vi "Claude_View.vi"(0 "State":T2={"Tick"=0, "Phase"=0, "PhaseTicks"=0, "Level"=1, "Room"=0, "X10"=0, "Y10"=0, "VY10"=0, "Mode"=0, "Facing"=0, "Run"=0, "Vert"=0, "StandY"=0, "EntryX10"=0, "EntryY10"=0, "EntryMode"=0, "Lives"=4, "Score"=0, "NextLife"=10000, "KeyR"=0, "KeyB"=0, "KeyY"=0, "Torch"=FALSE, "FloorPhase"=0, "Dead"=FALSE, "LevelStart"=FALSE, "Quit"=FALSE, "Sound"=0, "Seed"=12345, "DemoStep"=0, "Tiles"=[], "World"=[], "Enemies"=[], "Highscores"=[], "Name"=[0, 0, 0], "Cursor"=0}, 5 "Dark":bool) -> (4 "View":T1={"Hide"=FALSE, "CX"=0, "CY"=0, "ClaudeIdx"=-1, "ClaudeX"=0, "ClaudeY"=0})   [LabVIEW 2020, in "GH_Render.lvlib"]
doc: "What the drawing needs to know about Claude: his sprite (standing, walking, jumping, falling, climbing, sliding, dying with flashing; -1 on the title), his screen position, his tile (CX, CY, centre of the light circle) and Hide = Dark."
uses:
  GH_Render.lvlib
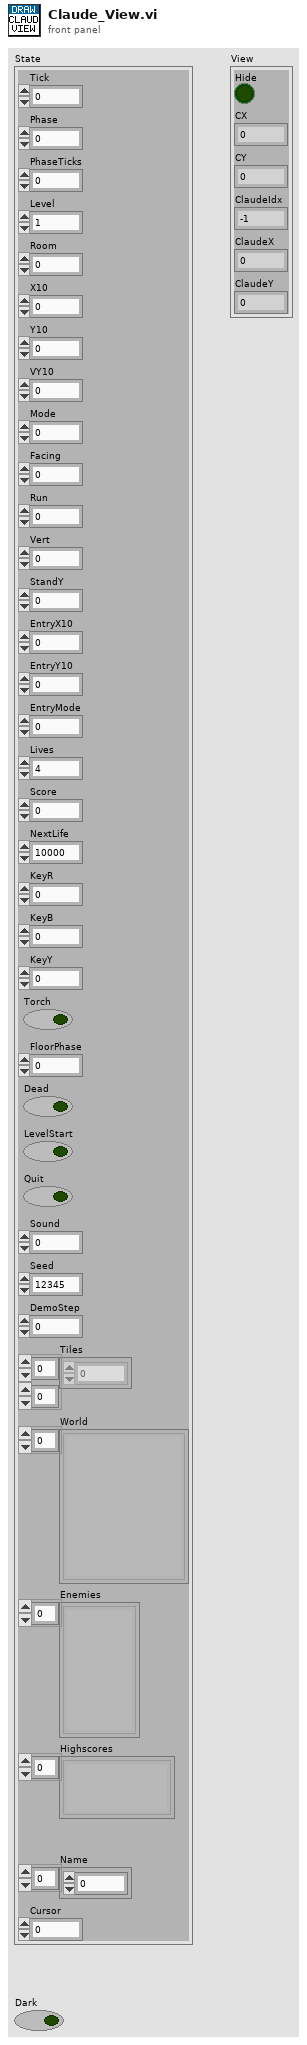
[diagram p1: front panel]
types:
  T1 = cluster{"Hide":bool, "CX":i32, "CY":i32, "ClaudeIdx":i32, "ClaudeX":i32, "ClaudeY":i32}
  T2 = cluster{"Tick":u32, "Phase":i32, "PhaseTicks":i32, "Level":i32, "Room":i32, "X10":i32, "Y10":i32, "VY10":i32, "Mode":i32, "Facing":i32, "Run":i32, "Vert":i32, "StandY":i32, "EntryX10":i32, "EntryY10":i32, "EntryMode":i32, "Lives":i32, "Score":i32, "NextLife":i32, "KeyR":i32, "KeyB":i32, "KeyY":i32, "Torch":bool, "FloorPhase":i32, "Dead":bool, "LevelStart":bool, "Quit":bool, "Sound":i32, "Seed":u32, "DemoStep":i32, "Tiles":u8[][], "World":cluster{"ID":string, "Depth":i32, "Column":i32, "Tiles":u8[][]}[], "Enemies":cluster{"Kind":i32, "X10":i32, "Y10":i32, "Dir":i32, "Mode":i32}[], "Highscores":cluster{"Score":i32, "Name":string}[], "Name":i32[], "Cursor":i32}
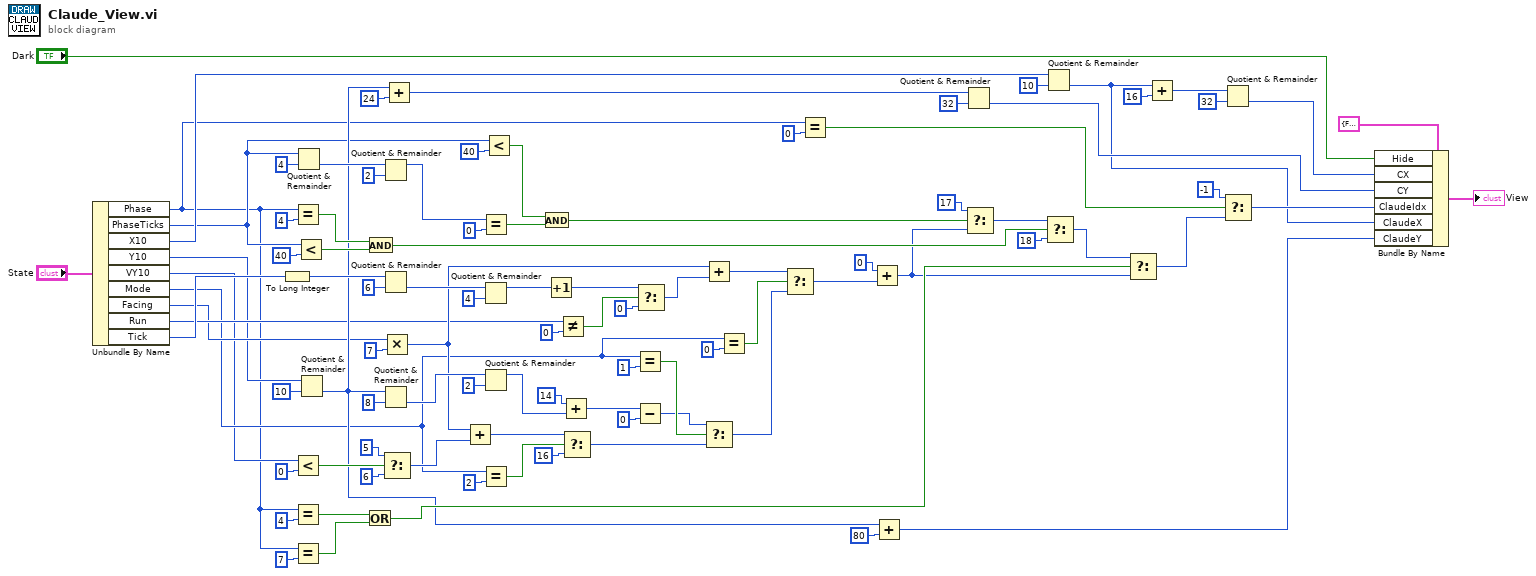
[diagram p0: block diagram]
diagram:
  n1 = Unbundle By Name("State") -> ("Phase"=w3:i32, "PhaseTicks"=w4:i32, "X10"=w5:i32, "Y10"=w6:i32, "VY10"=w7:i32, "Mode"=w8:i32, "Facing"=w9:i32, "Run"=w10:i32, "Tick"=w11:u32)
  n2 = To Long Integer(number=w11) -> (32bit integer=w28:i32)
  n3 = Equal?(x=w3, y=4) -> (x = y?=w80:bool)
  n4 = Less?(x=w7, y=0) -> (x < y?=w40:bool)
  n5 = Equal?(x=w3, y=4) -> (x = y?=w66:bool)
  n6 = Equal?(x=w3, y=7) -> (x = y?=w68:bool)
  n7 = Quotient & Remainder(x=w4, y=4) -> (floor(x/y)=w73:i32)  [unwired: 1 out]
  n8 = Less?(x=w4, y=40) -> (x < y?=w82:bool)
  n9 = Quotient & Remainder(x=w6, y=10) -> (floor(x/y)=w17:i32)  [unwired: 1 out]
  n10 = Or(x=w66, y=w68) -> (x .or. y?=w69:bool)
  n11 = And(x=w80, y=w82) -> (x .and. y?=w83:bool)
  n12 = Quotient & Remainder(x=w73, y=2) -> (x-y*floor(x/y)=w75:i32)  [unwired: 1 out]
  n13 = Quotient & Remainder(x=w28, y=6) -> (floor(x/y)=w30:i32)  [unwired: 1 out]
  n14 = Quotient & Remainder(x=w17, y=8) -> (floor(x/y)=w47:i32)  [unwired: 1 out]
  n15 = Multiply(x=w9, y=7) -> (x*y=w27:i32)
  n16 = Select(t=5, s=w40, f=6) -> (s? t:f=w43:i32)
  n17 = Add(x=w17, y=24) -> (x+y=w23:i32)
  n18 = Add(x=w27, y=w43) -> (x+y=w44:i32)
  n19 = Equal?(x=w75, y=0) -> (x = y?=w77:bool)
  n20 = Quotient & Remainder(x=w30, y=4) -> (x-y*floor(x/y)=w32:i32)  [unwired: 1 out]
  n21 = Quotient & Remainder(x=w47, y=2) -> (x-y*floor(x/y)=w49:i32)  [unwired: 1 out]
  n22 = Equal?(x=w8, y=2) -> (x = y?=w59:bool)
  n23 = Less?(x=w4, y=40) -> (x < y?=w71:bool)
  n24 = And(x=w71, y=w77) -> (x .and. y?=w78:bool)
  n25 = Increment(x=w32) -> (x+1=w33:i32)
  n26 = Not Equal?(x=w10, y=0) -> (x != y?=w35:bool)
  n27 = Add(x=14, y=w49) -> (x+y=w50:i32)
  n28 = Select(t=w44, s=w59, f=16) -> (s? t:f=w61:i32)
  n29 = Equal?(x=w8, y=1) -> (x = y?=w57:bool)
  n30 = Subtract(x=w50, y=0) -> (x-y=w52:i32)
  n31 = Select(t=w33, s=w35, f=0) -> (s? t:f=w37:i32)
  n32 = Add(x=w27, y=w37) -> (x+y=w38:i32)
  n33 = Select(t=w52, s=w57, f=w61) -> (s? t:f=w62:i32)
  n34 = Equal?(x=w8, y=0) -> (x = y?=w55:bool)
  n35 = Select(t=w38, s=w55, f=w62) -> (s? t:f=w63:i32)
  n36 = Equal?(x=w3, y=0) -> (x = y?=w13:bool)
  n37 = Add(x=0, y=w63) -> (x+y=w64:i32)
  n38 = Add(x=w17, y=80) -> (x+y=w93:i32)
  n39 = Quotient & Remainder(x=w23, y=32) -> (floor(x/y)=w25:i32)  [unwired: 1 out]
  n40 = Select(t=17, s=w78, f=w64) -> (s? t:f=w85:i32)
  n41 = Quotient & Remainder(x=w5, y=10) -> (floor(x/y)=w15:i32)  [unwired: 1 out]
  n42 = Select(t=w85, s=w83, f=18) -> (s? t:f=w87:i32)
  n43 = Select(t=w87, s=w69, f=w64) -> (s? t:f=w89:i32)
  n44 = Add(x=w15, y=16) -> (x+y=w19:i32)
  n45 = Quotient & Remainder(x=w19, y=32) -> (floor(x/y)=w21:i32)  [unwired: 1 out]
  n46 = Select(t=-1, s=w13, f=w89) -> (s? t:f=w90:i32)
  n47 = Bundle By Name(cluster=T1 {"Hide"=FALSE, "CX"=0, "CY"=0, "ClaudeIdx"=-1, "ClaudeX"=0, "ClaudeY"=0}, "Hide"="Dark", "CX"=w21, "CY"=w25, "ClaudeIdx"=w90, "ClaudeX"=w15, "ClaudeY"=w93) -> (→"View":T1)
